vi "FromRepo.vi"(8 "error in":errorcluster, 9 "from repo cluster":T2, 10 "repository in":refnum<class "NISE_CEF_Repository.lvclass">, 11 "node in":refnum<class "NISE_CEF_serializable node.lvclass">) -> (0 "error out":errorcluster, 2 "repository out":refnum<class "NISE_CEF_Repository.lvclass">, 3 "node":T1)   [LabVIEW 2014, in "NISE_CEF_serializable node.lvclass"]
doc: "Grabs information from the Repo and stores it in the nodes."
uses:
  NISE_CEF_serializable node.lvclass
  Repository/NISE_CEF_Repository.lvclass
  Node/FromRepoCluster.ctl
  Node/NodeRef.ctl
  Node/NISE_CEF_Node.lvclass
  hierarchy repo/NISE_CEF_HierarchyRepo.lvclass
  serializable configuration/NISE_CEF_serializable configuration.lvclass
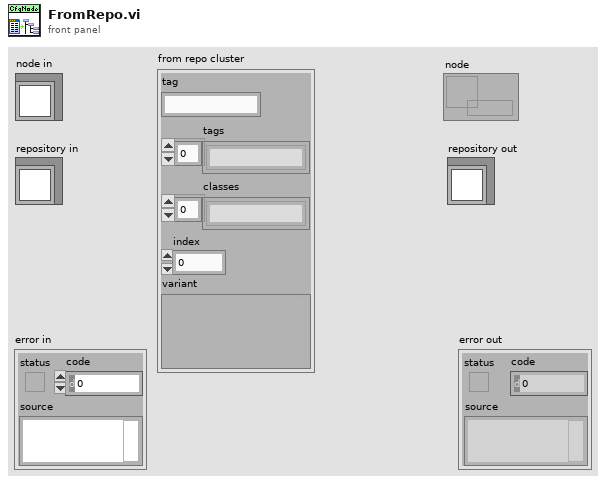
[diagram p1: front panel]
types:
  T1 = typedef "NISE_CEF_Node.lvclass/NodeRef.ctl" = refnum<data-value>
  T2 = typedef "NISE_CEF_Node.lvclass/FromRepoCluster.ctl" = cluster{"tag":string, "tags":string[], "classes":string[], "index":i32, "variant":variant}
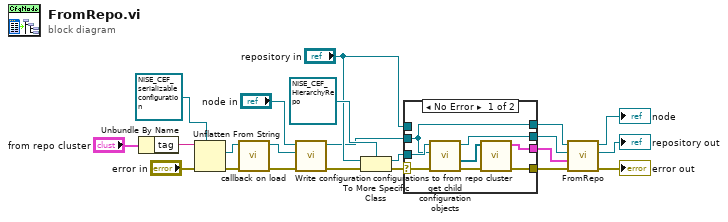
[diagram p0: block diagram]
diagram:
  n1 = Unbundle By Name("from repo cluster") -> ("tag"=w9:string)
  n2 = Unflatten From String(type=refnum<class "NISE_CEF_serializable configuration.lvclass"> refnum ("configuration"), binary string=w9, error in (no error)="error in") -> (value=w4:refnum<class "NISE_CEF_serializable configuration.lvclass">, error out=w3:errorcluster)  [unwired: 2 in, 1 out]
  n3 = call-dynamic "callback on load.vi"("error in"=w3, "configuration in"=w4) -> ("error out"=w2:errorcluster, "configuration out"=w1:refnum<class "NISE_CEF_serializable configuration.lvclass">)  [unwired: 8 in]
  n4 = call-dynamic "Write configuration.vi"("error in"=w2, "configuration"=w1, "NISE_CEF_serializable node in"="node in") -> ("error out"=w6:errorcluster, "NISE_CEF_serializable node out"=w5:refnum<class "NISE_CEF_serializable node.lvclass">)  [unwired: 7 in]
  n5 = To More Specific Class(target class=refnum<class "NISE_CEF_HierarchyRepo.lvclass"> refnum ("NISE_CEF_HierarchyRepo.lvclass"), reference="repository in", error in=w6) -> (specific class reference=w20:refnum<class "NISE_CEF_HierarchyRepo.lvclass">, error out=w22:errorcluster)
  n6 = case shown="No Error" w22 {
    selector: w22 -> [w28 w32]
    tunnel: "repository in" -> [_ w33]
    tunnel: [w29 w33] -> w17
    tunnel: [w25 w32] -> w19
    tunnel: w5 -> [w27 w31]
    tunnel: [w27 w31] -> w18
    tunnel: w20 -> [w30 _]
    tunnel: [w23 _] -> w12
    frame No Error {
      n7 = call-dynamic "get child configuration objects.vi"("error in"=w28, "serializable node"=w27, "NISE_CEF_HierarchyRepo in"=w30) -> ("error out"=w26:errorcluster, "children"=w24:refnum<class "NISE_CEF_serializable configuration.lvclass">[], "NISE_CEF_HierarchyRepo out"=w29:refnum<class "NISE_CEF_HierarchyRepo.lvclass">)  [unwired: 6 in]
      n8 = call "configurations to from repo cluster.vi"("error in"=w26, "configurations"=w24) -> ("error out"=w25:errorcluster, "from repo cluster"=w23:T2)  [unwired: 8 in]
    }
    frame Error {
    }
  }
  n9 = call-parent "FromRepo.vi"("error in"=w19, "from repo cluster"=w12, "repository in"=w17, "node in"=w18) -> ("error out"=→"error out":errorcluster, "repository out"=→"repository out":refnum<class "NISE_CEF_Repository.lvclass">, "node"=→"node":T1)  [unwired: 5 in]
